vi "Sample_IO_Task.vi"(8 "error in (no error)":errorcluster={"status"=FALSE, "code"=0, "source"="\"\""}, 9 "Tolerance":dbl=2.0, 10 "Flow SP":dbl=45.0, 11 "Pressure SP":dbl=100.0) -> (0 "error out":errorcluster, 2 "Condition Met":bool, 3 "Measured Pressure":dbl)   [LabVIEW 2026]
doc: "Worker task that reads plant feedback and evaluates step condition."
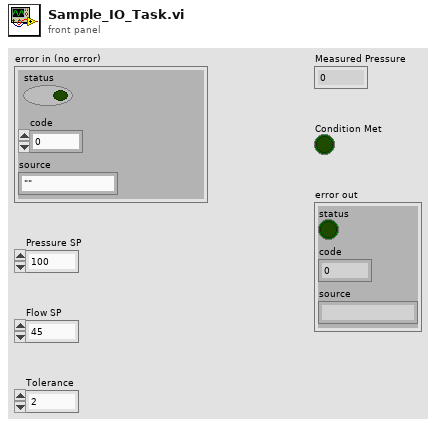
[diagram p1: front panel]
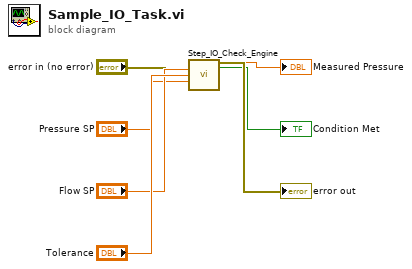
[diagram p0: block diagram]
diagram:
  n1 = call "Step_IO_Check_Engine.vi"("Target Flow SP (L/min)"="Flow SP", "Tolerance (bar)"="Tolerance", "error in (no error)"="error in (no error)", "Target Pressure SP (bar)"="Pressure SP") -> ("error out"=→"error out":errorcluster, "Condition Met"=→"Condition Met":bool, "Actual Pressure (bar)"=→"Measured Pressure":dbl)  [unwired: 7 in, 2 out]
